vi "Create LV File.vi"(6 "Output Folder":path, 8 "error in":errorcluster, 9 "Template":path, 10 "ILabVIEW File":refnum<class "ILabVIEW File.lvclass">, 11 "LV File Creator in":refnum<class "LV File Creator.lvclass">) -> (0 "error out":errorcluster, 2 "File Path":path, 3 "LV File Creator out":refnum<class "LV File Creator.lvclass">)   [LabVIEW 2026, in "LV File Creator.lvclass"]
doc: "Create labview file."
uses:
  LV File Creator.lvclass
  Interfaces/ILabVIEW File/ILabVIEW File.lvclass
  LV File Creator.lvclass/LV File Creator.ctl
  Interfaces/ILogger/ILogger Messages/Log Msg/Log Msg.lvclass/Log Msg.ctl
  <vilib>/ActorFramework/Message Enqueuer/Message Enqueuer.lvclass/Message Enqueuer.ctl
  <vilib>/ActorFramework/Message Enqueuer/Enqueue.vi
  Interfaces/ILogger/ILogger Messages/Log Msg/Log Msg.lvclass
  <vilib>/ActorFramework/Message Priority Queue/Priority Enqueue.vi
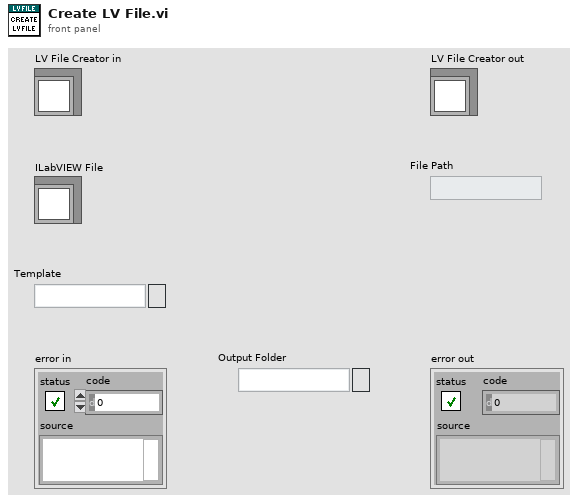
[diagram p1: front panel]
types:
  T1 = typedef "Log Entry--cluster.ctl" = cluster{"Time":timestamp, "Message":string}
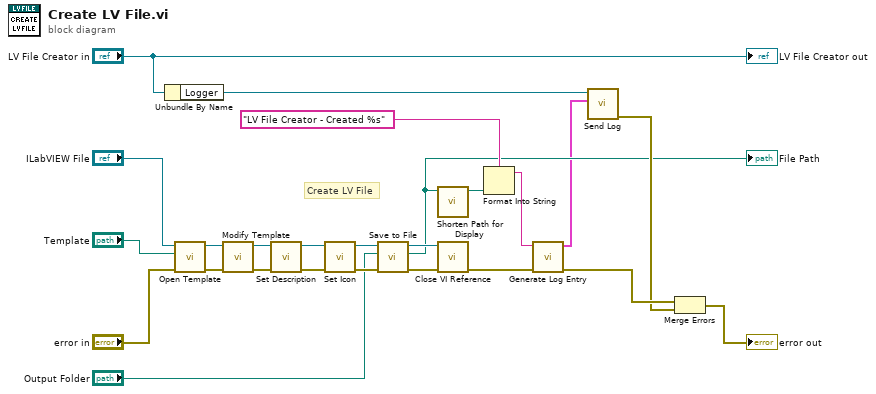
[diagram p0: block diagram]
diagram:
  # "Create LV File"
  n1 = Unbundle By Name("LV File Creator in") -> ("Logger"=w7:refnum<class "Message Enqueuer.lvclass">)
  n2 = call-dynamic "Open Template.vi"("error in"="error in", "Template"="Template", "ILabVIEWFile in"="ILabVIEW File") -> ("error out"=w25:errorcluster, "ILabVIEWFile out"=w15:refnum<class "ILabVIEW File.lvclass">)  [unwired: 7 in]
  n3 = call-dynamic "Modify Template.vi"("error in (no error)"=w25, "ILabVIEWFile in"=w15) -> ("error out"=w24:errorcluster, "ILabVIEWFile out"=w14:refnum<class "ILabVIEW File.lvclass">)  [unwired: 8 in]
  n4 = call-dynamic "Set Description.vi"("error in"=w24, "ILabVIEWFile in"=w14) -> ("error out"=w23:errorcluster, "ILabVIEWFile out"=w13:refnum<class "ILabVIEW File.lvclass">)  [unwired: 8 in]
  n5 = call-dynamic "Set Icon.vi"("error in"=w23, "ILabVIEWFile in"=w13) -> ("error out"=w22:errorcluster, "ILabVIEWFile out"=w12:refnum<class "ILabVIEW File.lvclass">)  [unwired: 8 in]
  n6 = call-dynamic "Save to File.vi"("error in"=w22, "Folder"="Output Folder", "ILabVIEWFile in"=w12) -> ("error out"=w21:errorcluster, "File Path"=w5:path, "ILabVIEWFile out"=w11:refnum<class "ILabVIEW File.lvclass">)  [unwired: 6 in]
  "File Path" <- w5
  n7 = call "Shorten Path for Display.vi"("Path"=w5) -> ("Shortened Path"=w4:path)  [unwired: 10 in]
  n8 = call-dynamic "Close VI Reference.vi"("error in"=w21, "ILabVIEWFile in"=w11) -> ("error out"=w19:errorcluster)  [unwired: 8 in, 1 out]
  n9 = Format Into String(format string="LV File Creator - Created %s", w4) -> (resulting string=w3:string)  [unwired: 2 in, 1 out]
  n10 = call "Generate Log Entry.vi"("error in"=w19, "Message"=w3) -> ("error out"=w18:errorcluster, "Log Entry"=w2:T1)  [unwired: 8 in]
  n11 = call "Send Log.vi"("Log Entry"=w2, "Message Enqueuer"=w7) -> ("error out"=w16:errorcluster)  [unwired: 8 in, 1 out]
  n12 = Merge Errors(w18, w16) -> (→"error out":errorcluster)
  "LV File Creator out" <- "LV File Creator in"
